vi "FuncVI-BPFilterBtw.vi"(5 "InstanceRef":T2, 9 "arg list":T1[](array[typedef]) {"num" format="%.2f"}) -> (0 "error out":bool, 3 "result":T1 {"num" format="%.2f"})   [LabVIEW 2021]
doc: "<B>FuncVI-BPFilterBtw</B>\n\nThis VI is example of implementation of CalcExpress function (FuncVI). The function implements <B>Bandpass Butterworth filter</B>.\n\n::: CalcExpress Toolkit :::\nCopyright (c) 2000-2026 Konstantin Shifershteyn. All rights reserved."
uses:
  vi.lib/addons/CalcExpress/cetypes.llb/CalcExpress Function Argument Info.ctl
  vi.lib/addons/CalcExpress/cetypes.llb/CalcExpress Instance RefNum.ctl
  <vilib>/Analysis/3filter.llb/Filter Passband Type.ctl
  <vilib>/Analysis/3filter.llb/IIR Cascade Filter with I.C. (DBL).vi
  <vilib>/Analysis/NI_AALBase.lvlib
panel:
  in  "max arg num":i32=6
  in  "min arg num":i32=4
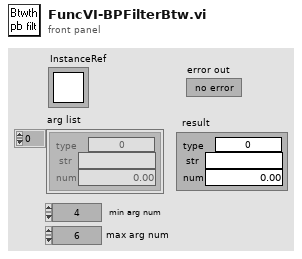
[diagram p1: front panel]
types:
  T1 = typedef "CalcExpress Function Argument Info.ctl" = cluster{"type":u32, "str":string, "num":dbl}
  T2 = typedef "CalcExpress Instance RefNum.ctl" = refnum<k1>
  T3 = enum32{"String", "DBL Number", "identifier", "1D Array of DBL", "2D Array of DBL", "CDB Number", "1D Array of CDB", "2D Array of CDB", "1D Array of String", "2D Array of String", "Unknown data type"}
  T4 = cluster{"index":i32, "data type":enum32{"String", "DBL Number", "identifier", "1D Array of DBL", "2D Array of DBL", "CDB Number", "1D Array of CDB", "2D Array of CDB", "1D Array of String", "2D Array of String", "Unknown data type"}, "default num":dbl, "default str":string}[]
  T5 = typedef "NI_AALBase.lvlib/Filter Passband Type.ctl" = enum32{"Lowpass", "Highpass", "Bandpass", "Bandstop"}
  T6 = typedef "VarMan Variable Context Handle.ctl" = i32
  T7 = cluster{"filter structure":enum32{"IIR 2nd Order", "IIR 4th Order"}, "Reverse Coefficients":dbl[], "Forward Coefficients":dbl[]}
  T8 = cluster{"data type":enum32{"String", "DBL Number", "identifier", "1D Array of DBL", "2D Array of DBL", "CDB Number", "1D Array of CDB", "2D Array of CDB", "1D Array of String", "2D Array of String", "Unknown data type"}, "data string":string, dbl}
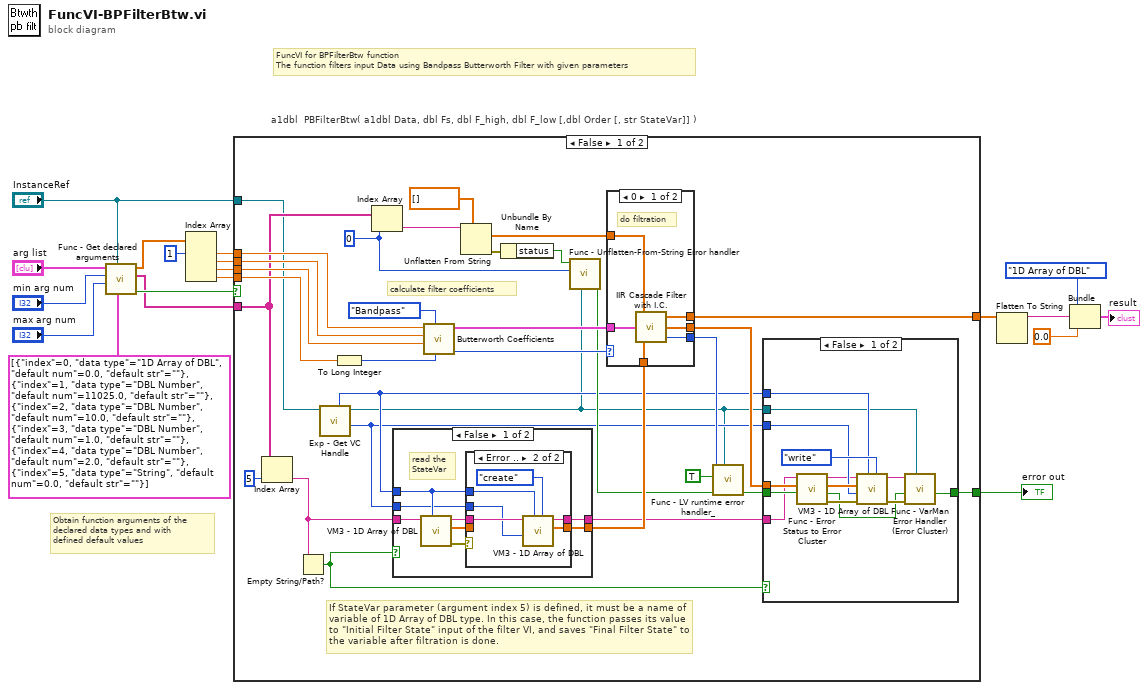
[diagram p0: block diagram]
diagram:
  # "FuncVI for BPFilterBtw function\nThe function filters input Data using Bandpass Butterworth Filter with given parameters"
  # "Obtain function arguments of the\ndeclared data types and with\ndefined default values"
  # "a1dbl  PBFilterBtw( a1dbl Data, dbl Fs, dbl F_high, dbl F_low [,dbl Order [, str StateVar]] )"
  n1 = call "Func - Get declared arguments.vi"("arg descriptors"=T4 [{"index"=0, "data type"=enum."1D Array of DBL", "default num"=0.0, "default str"=""}, {"index"=1, "data type"=enum."DBL Number", "default num"=11025.0, "default str"=""}, {"index"=2, "data type"=enum."DBL Number", "default num"=10.0, "default str"=""}, {"index"=3, "data type"=enum."DBL Number", "default num"=1.0, "default str"=""}, {"index"=4, "data type"=enum."DBL Number", "default num"=2.0, "default str"=""}, {"index"=5, "data type"=enum."String", "default num"=0.0, "default str"=""}] ("args descriptors"), "InstanceRef"="InstanceRef", "max arg num"="max arg num", "min arg num"="min arg num", "arg list"="arg list") -> ("error out"=w17:bool, "str list"=w9:string[], "num list"=w6:dbl[])  [unwired: 3 in, 1 out]
  n2 = Index Array(array=w6, index #1=1 ("index")) -> (element #1=w4:dbl, element #2=w3:dbl, element #3=w2:dbl, element #4=w1:dbl)  [unwired: 3 in]
  n3 = case shown="False" w17 {
    selector: w17 -> [_ w89]
    tunnel: [w36 w89] -> w16
    tunnel: "InstanceRef" -> [w22 _]
    tunnel: w4 -> [w50 _]
    tunnel: w3 -> [w49 _]
    tunnel: w2 -> [w48 _]
    tunnel: w1 -> [w47 _]
    tunnel: [w42 _] -> w11
    tunnel: w9 -> [w39 _]
    frame False {
      w31 = 0
      # "If StateVar parameter (argument index 5) is defined, it must be a name of\nvariable of 1D Array of DBL type. In this case, the function passes its value\nto \"Initial Filter State\" input of the filter VI, and saves \"Final Filter State\" to\nthe variable after filtration is done."
      # "calculate filter coefficients"
      n4 = Index Array(array=w39, index=5) -> (element=w27:string)
      n5 = Empty String/Path?(string/path=w27) -> (empty?=w28:bool)
      n6 = call "Exp - Get VC Handle.vi"("InstanceRef"=w22) -> ("writer ID"=w25:u32, "dup InstanceRef"=w23:T2, "VC Handle"=w26:T6)  [unwired: 5 in, 1 out]
      n7 = To Long Integer(number=w47) -> (32bit integer=w46:i32)
      n8 = Index Array(array=w39, index=w31) -> (element=w41:string)
      n9 = case shown="False" w28 {
        tunnel: [w67 _] -> w38
        tunnel: w27 -> [w71 w80]
        tunnel: w25 -> [w64 _]
        tunnel: w26 -> [w65 _]
        tunnel: [w69 w80] -> w24
        frame False {
          # "read the\nStateVar"
          n10 = call "VM3 - 1D Array of DBL.vi"("VC Handle"=w65, "name_spec"=w71) -> ("error out"=w70:errorcluster, "value out"=w66:dbl[], "dup name_spec"=w68:string)  [unwired: 6 in, 1 out]
          n11 = case shown="Error .." w70 {
            tunnel: [w73 w78] -> w69
            tunnel: w68 -> [w73 w79]
            tunnel: [w72 w77] -> w67
            tunnel: w66 -> [w72 _]
            tunnel: w65 -> [_ w76]
            tunnel: w64 -> [_ w75]
            frame No Error {
            }
            frame Error {
              n12 = call "VM3 - 1D Array of DBL.vi"("cmd (read)"=enum16{"create", "destroy", "write", "read"}."create", "VC Handle"=w76, "writer ID"=w75, "name_spec"=w79) -> ("value out"=w77:dbl[], "dup name_spec"=w78:string)  [unwired: 4 in, 2 out]
            }
          }
        }
        frame True {
        }
      }
      n13 = call <vilib>:"Butterworth Coefficients.vi"("order"=w46, "filter type"=Filter_Passband_Type."Bandpass", "low cutoff freq: fl"=w48, "high cutoff freq: fh"=w49, "sampling freq: fs"=w50) -> ("error"=w45:i32, "IIR Filter Cluster"=w44:T7)  [unwired: 5 in]
      n14 = Unflatten From String(type=dbl[] [], binary string=w41) -> (value=w43:dbl[], error out=w29:errorcluster)  [unwired: 3 in, 1 out]
      n15 = Unbundle By Name(w29) -> ("status"=w32:bool)
      n16 = call "Func - Unflatten-From-String Error handler.vi"("InstanceRef"=w23, "argument number"=w31, "Unflatten Error status"=w32) -> ("error out"=w30:bool)  [unwired: 6 in]
      n17 = case shown="0" w45 {
        selector: w45 -> [_ w88]
        tunnel: w44 -> [w86 _]
        tunnel: [w85 w88] -> w35
        tunnel: [w84 _] -> w42
        tunnel: [w83 w87] -> w37
        tunnel: w38 -> [w82 w87]
        tunnel: w43 -> [w81 _]
        frame 0 {
          # "do filtration"
          n18 = call-poly <vilib>:"IIR Cascade Filter with I.C..vi"("Initial Filter State"=w82, "IIR Filter Cluster"=w86, "X"=w81) -> ("error"=w85:i32, "Final Filter State"=w83:dbl[], "Filtered X"=w84:dbl[])
        }
        frame Default {
        }
      }
      n19 = call "Func - LV runtime error handler_.vi"("InstanceRef"=w23, "error in"=w30, "Gen CE error?"=TRUE, "LabVIEW error code"=w35) -> ("error out"=w33:bool)  [unwired: 7 in]
      n20 = case shown="False" w28 {
        tunnel: w37 -> [w55 _]
        tunnel: [w56 w63] -> w36
        tunnel: w33 -> [w57 w63]
        tunnel: w26 -> [w54 _]
        tunnel: w25 -> [w53 _]
        tunnel: w24 -> [w52 _]
        tunnel: w23 -> [w51 _]
        frame False {
          n21 = call "Func - Error Status to Error Cluster.vi"("error status in"=w57) -> ("Error Cluster out"=w60:errorcluster, "error status out"=w59:bool)  [unwired: 9 in]
          n22 = call "VM3 - 1D Array of DBL.vi"("cmd (read)"=enum16{"create", "destroy", "write", "read"}."write", "VC Handle"=w54, "error in"=w60, "writer ID"=w53, "value in"=w55, "name_spec"=w52) -> ("error out"=w61:errorcluster, "dup name_spec"=w62:string)  [unwired: 2 in, 2 out]
          n23 = call "Func - VarMan Error Handler (Error Cluster).vi"("InstanceRef"=w51, "VarMan VI error in"=w61, "error status before"=w59, "var name"=w62) -> ("FuncVI error out"=w56:bool)  [unwired: 5 in, 2 out]
        }
        frame True {
        }
      }
    }
    frame True {
    }
  }
  "error out" <- w16
  n24 = Flatten To String(anything=w11) -> (data string=w10:string)  [unwired: 3 in, 2 out]
  n25 = Bundle("data type"=T3."1D Array of DBL", "data string"=w10, 0.0) -> (→"result":T8)  [unwired: 1 in]
